vi "Cleanup Channels.vi"(8 "error in (no error)":errorcluster, 11 "Plugin In":refnum<class "Sequencer with Output Values.lvclass">) -> (0 "error out":errorcluster, 1 "Num of Digital Channels":i32, 2 "Num of Analog Channels":i32, 3 "Plugin out":refnum<class "Sequencer with Output Values.lvclass">)   [LabVIEW 2024, in "Sequencer with Output Values.lvlib" / "Sequencer with Output Values.lvclass"]
uses:
  Sequencer with Output Values.lvclass
  C:/Program Files/National Instruments/LabVIEW 2024/vi.lib/FlexLogger/SDK/PluginSDK.lvlibp/PEFClasses/SDK/Plugin/Plugin.lvclass
  <vilib>/FlexLogger/SDK/PluginSDK.lvlibp/PEFClasses/SDK/Channel/Data Type_v2.ctl
  Sequencer with Output Values.lvclass/Sequencer with Output Values.ctl
  Global Strings.vi
  <vilib>/FlexLogger/SDK/PluginSDK.lvlibp/PEFClasses/SDK/Plugin/Read Channels.vi
  <vilib>/FlexLogger/SDK/PluginSDK.lvlibp/PEFClasses/SDK/Channel/Channel.lvclass
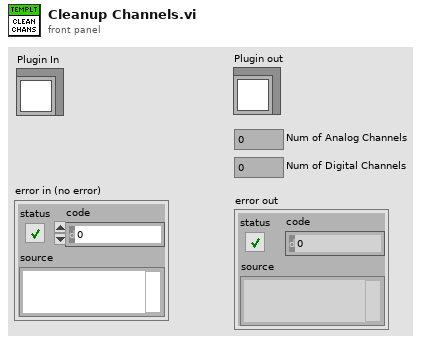
[diagram p1: front panel]
types:
  T1 = typedef "PluginSDK.lvlibp/Channel.lvclass/Data Type_v2.ctl" = u16
  T2 = typedef "Sequencer with Output Values.lvlib/Sequencer with Output Values.lvclass/Params.ctl" = cluster{"Step Values":T3[], "Only Execute When Test Running":bool, "Reset Sequence When Test Starts":bool, "Current Sequence ID":u32, "Total Iterations":u32, "Current Step Start Timestamp":dbl, "Number of Sequence Steps":i32, "Num of Analog Channels":i32, "Num of Digital Channels":i32, "Delay Before Starting Sequence":dbl, "Show UI":bool, "Time Remaining":dbl, "Test Running":bool, "Pause Timestamp":dbl, "Default Analog Values":dbl[], "Default Digital Values":bool[]}
  T3 = typedef "Sequencer with Output Values.lvlib/Sequencer with Output Values.lvclass/Step Settings.ctl" = cluster{"Duration":dbl, "Mode":string, "Delay Between Values":dbl, "Analog Values":string[], "Digital Values":string[]}
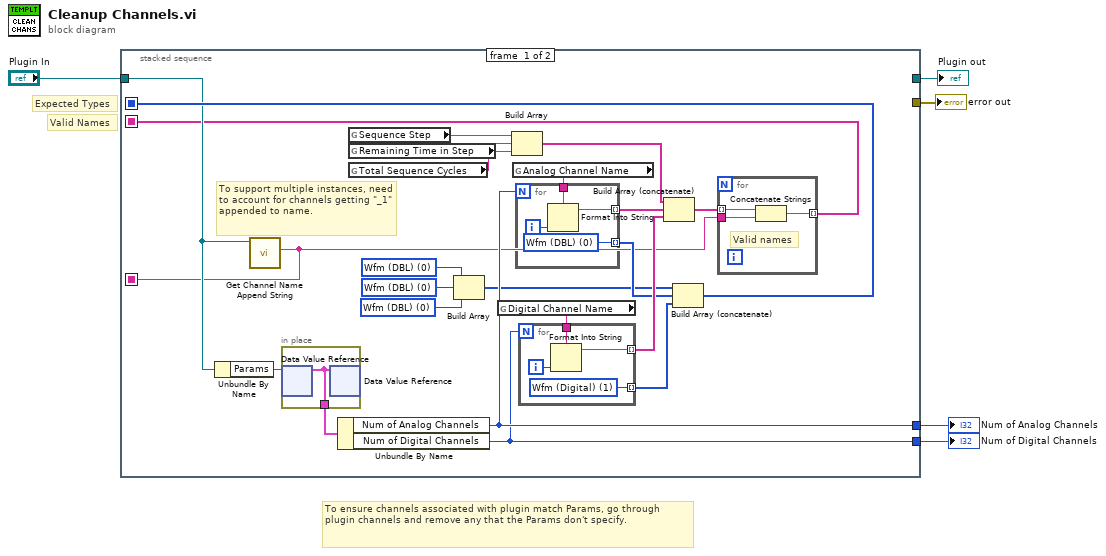
[diagram p0: block diagram]
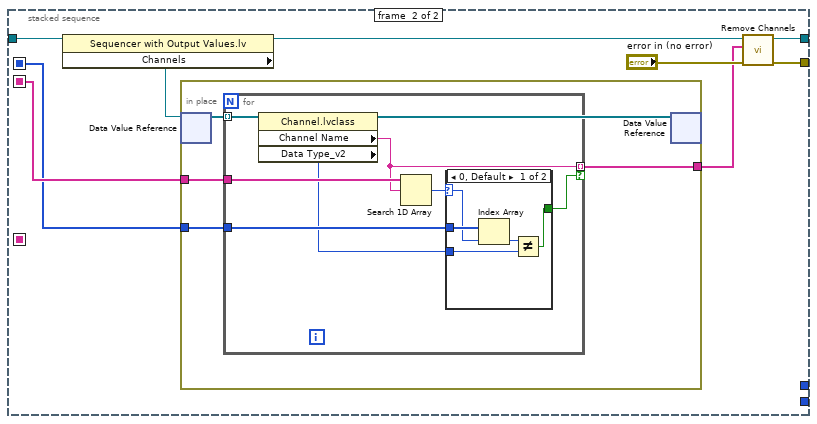
[diagram p2: hidden frame]
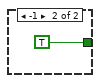
[diagram p3: hidden frame]
diagram:
  # "Expected Types"
  # "Valid Names"
  # "To ensure channels associated with plugin match Params, go through plugin channels and remove any that the Params don't specify."
  n1 = stacked-sequence {
    seq-local: [w7 _] -> [_ w47]
    seq-local: [w10 _] -> [_ w44]
    seq-local: [w6 _] -> [_ _]
    tunnel: [w22 _] -> w5
    tunnel: "Plugin In" -> [w8 w43]
    tunnel: [w26 _] -> w3
    tunnel: [_ w41] -> w2
    tunnel: [_ w45] -> w1
    frame #0 {
      w13 = T1 0 items=["Wfm (DBL)", "Wfm (Digital)", "String"] ("Data Type_v2")
      w14 = T1 0 items=["Wfm (DBL)", "Wfm (Digital)", "String"] ("Data Type_v2")
      w15 = T1 0 items=["Wfm (DBL)", "Wfm (Digital)", "String"] ("Data Type_v2")
      # "To support multiple instances, need to account for channels getting \"_1\" appended to name."
      n2 = Unbundle By Name(w8) -> ("Params"=w27:refnum<data-value>)
      n3 = call "Get Channel Name Append String.vi"("Plugin In"=w8) -> ("Channel Append String"=w6:string)  [unwired: 8 in, 2 out]
      n4 = in-place {
        in-place-border: [w40] -> w28
        n5 = in-place-dvr #1(w27) -> (w40:T2)  [unwired: 1 out]
        n6 = in-place-dvr #1(w40) -> ()  [unwired: 2 out]
      }
      n7 = Unbundle By Name(w28) -> ("Num of Analog Channels"=w26:i32, "Num of Digital Channels"=w22:i32)
      n8 = global read "Global Strings.vi" "Sequence Step"() -> (w21:string)
      n9 = global read "Global Strings.vi" "Remaining Time in Step"() -> (w20:string)
      n10 = global read "Global Strings.vi" "Total Sequence Cycles"() -> (w19:string)
      n11 = Build Array(w15, w14, w13) -> (w12:T1[])
      n12 = global read "Global Strings.vi" "Digital Channel Name"() -> (w24:string)
      n13 = Build Array(w21, w20, w19) -> (w18:string[])
      n14 = global read "Global Strings.vi" "Analog Channel Name"() -> (w25:string)
      n15 = for {
        N: w26 -> [_]
        tunnel: w25 -> [w38]
        tunnel: [w37] -> w23 mode=indexing
        tunnel: [w36] -> w16 mode=indexing
        i -> [w39]
        w36 = T1 0 items=["Wfm (DBL)", "Wfm (Digital)", "String"] ("Data Type_v2")
        n16 = Format Into String(format string=w38, w39) -> (resulting string=w37:string)  [unwired: 2 in, 1 out]
      }
      n17 = for {
        N: w22 -> [_]
        tunnel: w24 -> [w34]
        tunnel: [w33] -> w17 mode=indexing
        tunnel: [w32] -> w11 mode=indexing
        i -> [w35]
        w32 = T1 1 items=["Wfm (DBL)", "Wfm (Digital)", "String"] ("Data Type_v2")
        n18 = Format Into String(format string=w34, w35) -> (resulting string=w33:string)  [unwired: 2 in, 1 out]
      }
      n19 = Build Array (concatenate)(w18, w23, w17) -> (w9:string[])
      n20 = Build Array (concatenate)(w12, w16, w11) -> (w10:T1[])
      n21 = for {
        tunnel: w9 -> [w31] mode=indexing
        tunnel: w6 -> [w30]
        tunnel: [w29] -> w7 mode=indexing
        # "Valid names"
        n22 = Concatenate Strings(w31, w30) -> (w29:string)
      }
    }
    frame #1 {
      n23 = property class="Sequencer with Output Values.lv"(reference=w43) -> (reference out=w49:refnum<class "Sequencer with Output Values.lvclass">, "Channels"=w48:refnum<data-value>)  [unwired: 1 in, 1 out]
      n24 = in-place {
        in-place-border: [w52] -> w42
        in-place-border: w47 -> [w51]
        in-place-border: w44 -> [w50]
        n25 = in-place-dvr #2(w48) -> (w53:refnum<class "Channel.lvclass">[])  [unwired: 1 out]
        n26 = for {
          tunnel: w53 -> [w60] mode=indexing
          tunnel: [w58] -> w52 mode=indexing if=w56
          tunnel: w51 -> [w59]
          tunnel: w50 -> [w55]
          n27 = property class="Channel.lvclass"(reference=w60) -> ("Channel Name"=w58:string, "Data Type_v2"=w54:T1)  [unwired: 1 in, 2 out]
          n28 = Search 1D Array(1D array=w59, element=w58) -> (index of element=w57:i32)  [unwired: 1 in]
          n29 = case shown="0, Default" w57 {
            selector: w57 -> [w64 _]
            tunnel: [w61 TRUE] -> w56
            tunnel: w55 -> [w65 _]
            tunnel: w54 -> [w62 _]
            frame 0, Default {
              n30 = Index Array(array=w65, index=w64) -> (element=w63:T1)
              n31 = Not Equal?(x=w63, y=w62) -> (x != y?=w61:bool)
            }
            frame -1 {
            }
          }
        }
        n32 = in-place-dvr #2(w53) -> ()  [unwired: 2 out]
      }
      n33 = call-dynamic "Remove Channels.vi"("error in (no error)"="error in (no error)", "Unique Channel Identifiers to Delete"=w42, "Plugin in"=w49) -> ("error out"=w41:errorcluster, "Plugin out"=w45:refnum<class "Sequencer with Output Values.lvclass">)  [unwired: 7 in]
    }
  }
  "Num of Analog Channels" <- w3
  "Num of Digital Channels" <- w5
  "error out" <- w2
  "Plugin out" <- w1
